vi "Ecrire regulateur MODBUS EPC3000.vi"(2 "Config + programmes":T1, 4 "Adresse régulateur":u8=1 min=1 max=16 step=1, 5 "Port COM run 1 REG":refnum<visa-resource-name>) -> (0 "error IO":errorcluster)   [LabVIEW 2022 SP3]
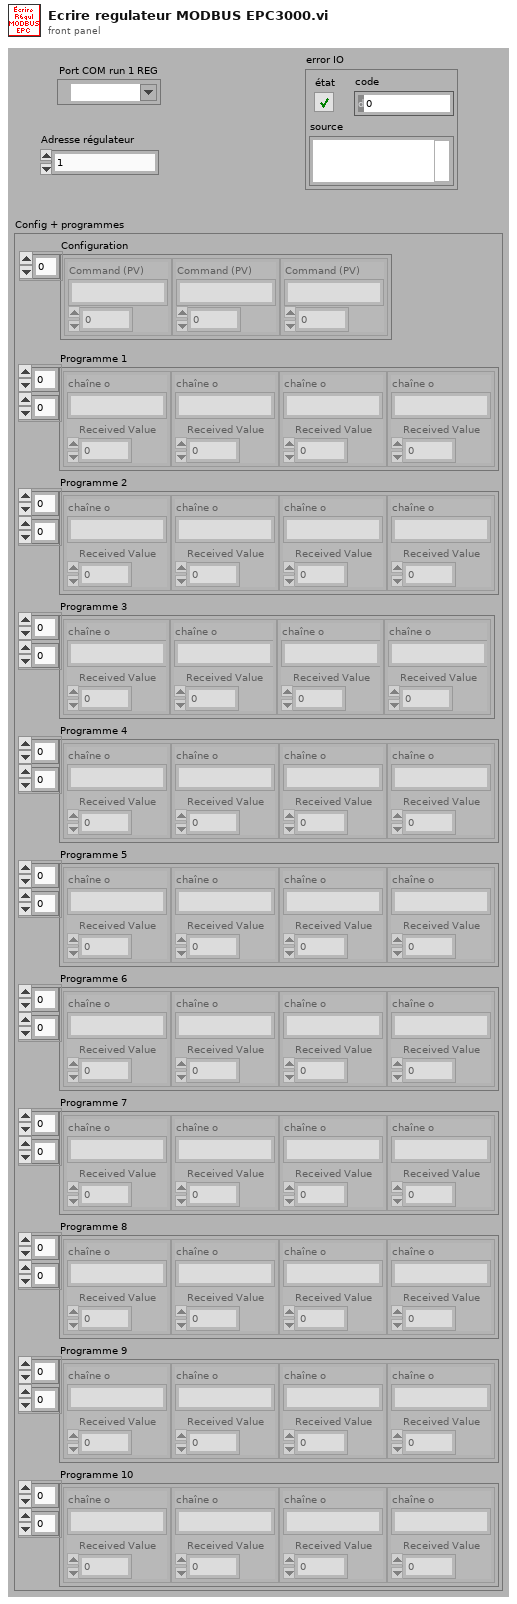
[diagram p1: front panel]
types:
  T1 = cluster{"Configuration":cluster{"Command (PV)":string, dbl}[], "Programme 1":cluster{"chaîne o":string, "Received Value":dbl}[][], "Programme 2":cluster{"chaîne o":string, "Received Value":dbl}[][], "Programme 3":cluster{"chaîne o":string, "Received Value":dbl}[][], "Programme 4":cluster{"chaîne o":string, "Received Value":dbl}[][], "Programme 5":cluster{"chaîne o":string, "Received Value":dbl}[][], "Programme 6":cluster{"chaîne o":string, "Received Value":dbl}[][], "Programme 7":cluster{"chaîne o":string, "Received Value":dbl}[][], "Programme 8":cluster{"chaîne o":string, "Received Value":dbl}[][], "Programme 9":cluster{"chaîne o":string, "Received Value":dbl}[][], "Programme 10":cluster{"chaîne o":string, "Received Value":dbl}[][]}
  T2 = cluster{"chaîne o":string, "Received Value":dbl}[][]
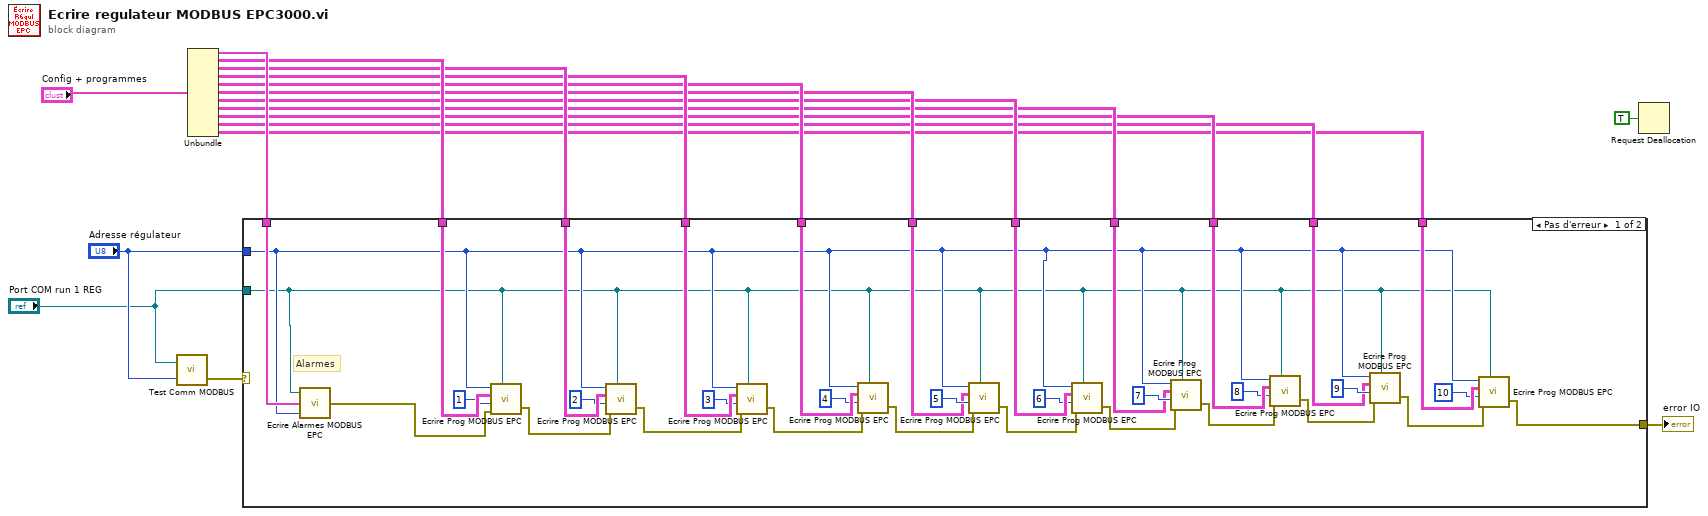
[diagram p0: block diagram]
diagram:
  n1 = call "Test Comm MODBUS.vi"("Adresse rég"="Adresse régulateur", "Port COM run 1 REG"="Port COM run 1 REG") -> ("error out"=w9:errorcluster)  [unwired: 1 in]
  n2 = Unbundle("Config + programmes") -> ("Configuration"=w15:cluster{"Command (PV)":string, dbl}[], "Programme 1"=w14:T2, "Programme 2"=w13:T2, "Programme 3"=w12:T2, "Programme 4"=w11:T2, "Programme 5"=w6:T2, "Programme 6"=w5:T2, "Programme 7"=w4:T2, "Programme 8"=w3:T2, "Programme 9"=w2:T2, "Programme 10"=w1:T2)
  n3 = case shown="Pas d'erreur" w9 {
    selector: w9 -> [_ w52]
    tunnel: "Adresse régulateur" -> [w27 _]
    tunnel: [w19 w52] -> w8
    tunnel: w15 -> [w51 _]
    tunnel: w14 -> [w50 _]
    tunnel: w13 -> [w49 _]
    tunnel: w12 -> [w48 _]
    tunnel: w11 -> [w47 _]
    tunnel: "Port COM run 1 REG" -> [w26 _]
    tunnel: w6 -> [w38 _]
    tunnel: w5 -> [w37 _]
    tunnel: w4 -> [w34 _]
    tunnel: w3 -> [w33 _]
    tunnel: w2 -> [w30 _]
    tunnel: w1 -> [w29 _]
    frame No Error {
      # "Alarmes"
      n4 = call "Ecrire Alarmes MODBUS EPC.vi"("Adresse rég"=w27, "Programmation configuration"=w51, "Port COM run 1 REG"=w26) -> ("error out"=w18:errorcluster)
      n5 = call "Ecrire Prog MODBUS EPC.vi"("Adresse rég"=w27, "Programme"=w50, "N° prog"=u16 1 ("Numéro de programme"), "error in"=w18, "Port COM run 1 REG"=w26) -> ("error out"=w46:errorcluster)  [unwired: 1 in]
      n6 = call "Ecrire Prog MODBUS EPC.vi"("Adresse rég"=w27, "Programme"=w49, "N° prog"=u16 2 ("Numéro de programme"), "error in"=w46, "Port COM run 1 REG"=w26) -> ("error out"=w44:errorcluster)  [unwired: 1 in]
      n7 = call "Ecrire Prog MODBUS EPC.vi"("Adresse rég"=w27, "Programme"=w48, "N° prog"=u16 3 ("Numéro de programme"), "error in"=w44, "Port COM run 1 REG"=w26) -> ("error out"=w43:errorcluster)  [unwired: 1 in]
      n8 = call "Ecrire Prog MODBUS EPC.vi"("Adresse rég"=w27, "Programme"=w47, "N° prog"=u16 4 ("Numéro de programme"), "error in"=w43, "Port COM run 1 REG"=w26) -> ("error out"=w25:errorcluster)  [unwired: 1 in]
      n9 = call "Ecrire Prog MODBUS EPC.vi"("Adresse rég"=w27, "Programme"=w38, "N° prog"=u16 5 ("Numéro de programme"), "error in"=w25, "Port COM run 1 REG"=w26) -> ("error out"=w24:errorcluster)  [unwired: 1 in]
      n10 = call "Ecrire Prog MODBUS EPC.vi"("Adresse rég"=w27, "Programme"=w37, "N° prog"=u16 6 ("Numéro de programme"), "error in"=w24, "Port COM run 1 REG"=w26) -> ("error out"=w23:errorcluster)  [unwired: 1 in]
      n11 = call "Ecrire Prog MODBUS EPC.vi"("Adresse rég"=w27, "Programme"=w34, "N° prog"=u16 7 ("Numéro de programme"), "error in"=w23, "Port COM run 1 REG"=w26) -> ("error out"=w22:errorcluster)  [unwired: 1 in]
      n12 = call "Ecrire Prog MODBUS EPC.vi"("Adresse rég"=w27, "Programme"=w33, "N° prog"=u16 8 ("Numéro de programme"), "error in"=w22, "Port COM run 1 REG"=w26) -> ("error out"=w21:errorcluster)  [unwired: 1 in]
      n13 = call "Ecrire Prog MODBUS EPC.vi"("Adresse rég"=w27, "Programme"=w30, "N° prog"=u16 9 ("Numéro de programme"), "error in"=w21, "Port COM run 1 REG"=w26) -> ("error out"=w20:errorcluster)  [unwired: 1 in]
      n14 = call "Ecrire Prog MODBUS EPC.vi"("Adresse rég"=w27, "Programme"=w29, "N° prog"=u16 10 ("Numéro de programme"), "error in"=w20, "Port COM run 1 REG"=w26) -> ("error out"=w19:errorcluster)  [unwired: 1 in]
    }
    frame Error {
    }
  }
  "error IO" <- w8
  n15 = Request Deallocation(TRUE ("flag")) -> ()
